vi "test scale by two.vi"(8 "error in (no error)":errorcluster, 11 "TestCase in":refnum<class "Scale Tests.lvclass">) -> (0 "error out":errorcluster, 3 "TestCase out":refnum<class "Scale Tests.lvclass">)   [LabVIEW 2026, in "Scale Tests.lvclass"]
doc: "Scale By Two.vi doubles 21 to 42."
uses:
  Scale Tests.lvclass
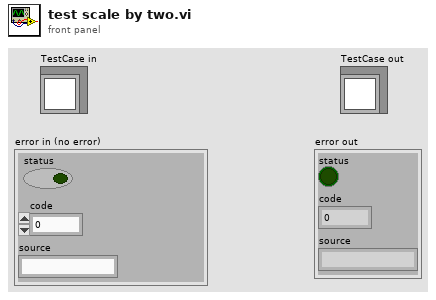
[diagram p1: front panel]
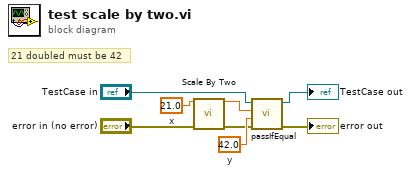
[diagram p0: block diagram]
diagram:
  w6 = 42.0  # y
  w3 = 21.0  # x
  # "21 doubled must be 42"
  n1 = call "Scale By Two.vi"("x"=w3, "error in"="error in (no error)") -> ("x times two"=w4:dbl, "error out"=w5:errorcluster)  [unwired: 12 in]
  n2 = call-dynamic "passIfEqual.vi"("error in (no error)"=w5, "y"=w6, "x"=w4, "TestCase in"="TestCase in") -> ("error out"=→"error out":errorcluster, "TestCase out"=→"TestCase out":refnum<class "Scale Tests.lvclass">)  [unwired: 6 in]
